vi "Combo Box Probe.vi"(0 "Abort Code":string(combo)="0503 0000h – Toggle bit not alternated.", 11 "error in":errorcluster) -> (4 "Items":string[](array[string]), 6 "Text":string(combo), 15 "error out":errorcluster)   [LabVIEW 2026]
doc: "Combo box probe – reads its own items."
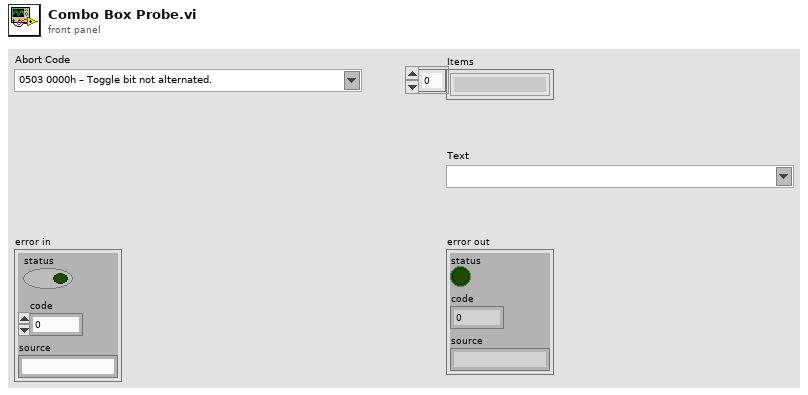
[diagram p1: front panel]
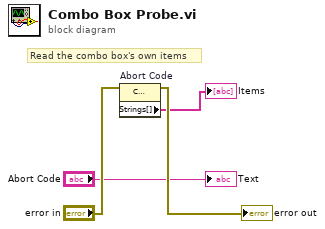
[diagram p0: block diagram]
diagram:
  # "Read the combo box's own items"
  n1 = property on="Abort Code" class="CmbBox"(error in="error in") -> (error out=→"error out":errorcluster, "Strings[]"=→"Items":string[])  [unwired: 1 in, 1 out]
  "Text" <- "Abort Code"
